vi "Claude_Blit.vi"(0 "Picture":u8[][](array[numeric]), 5 "Sprites":cluster{"Pix":u8[][], "Mask":u8[][]}[](array[cluster]), 7 "State":T2={"Tick"=0, "Phase"=0, "PhaseTicks"=0, "Level"=1, "Room"=0, "X10"=0, "Y10"=0, "VY10"=0, "Mode"=0, "Facing"=0, "Run"=0, "Vert"=0, "StandY"=0, "EntryX10"=0, "EntryY10"=0, "EntryMode"=0, "Lives"=4, "Score"=0, "NextLife"=10000, "KeyR"=0, "KeyB"=0, "KeyY"=0, "Torch"=FALSE, "FloorPhase"=0, "Dead"=FALSE, "LevelStart"=FALSE, "Quit"=FALSE, "Sound"=0, "Seed"=12345, "DemoStep"=0, "Tiles"=[], "World"=[], "Enemies"=[], "Highscores"=[], "Name"=[0, 0, 0], "Cursor"=0}, 9 "View":T1={"Hide"=FALSE, "CX"=0, "CY"=0, "ClaudeIdx"=-1, "ClaudeX"=0, "ClaudeY"=0}, 11 "error in":errorcluster) -> (4 "Picture out":u8[][](array[numeric]), 15 "error out":errorcluster)   [LabVIEW 2020, in "GH_Render.lvlib"]
doc: "Draws Claude (View: ClaudeIdx < 0 hides him) into the screen raster and, while he falls in the treasure room, the parachute above him."
uses:
  GH_Render.lvlib
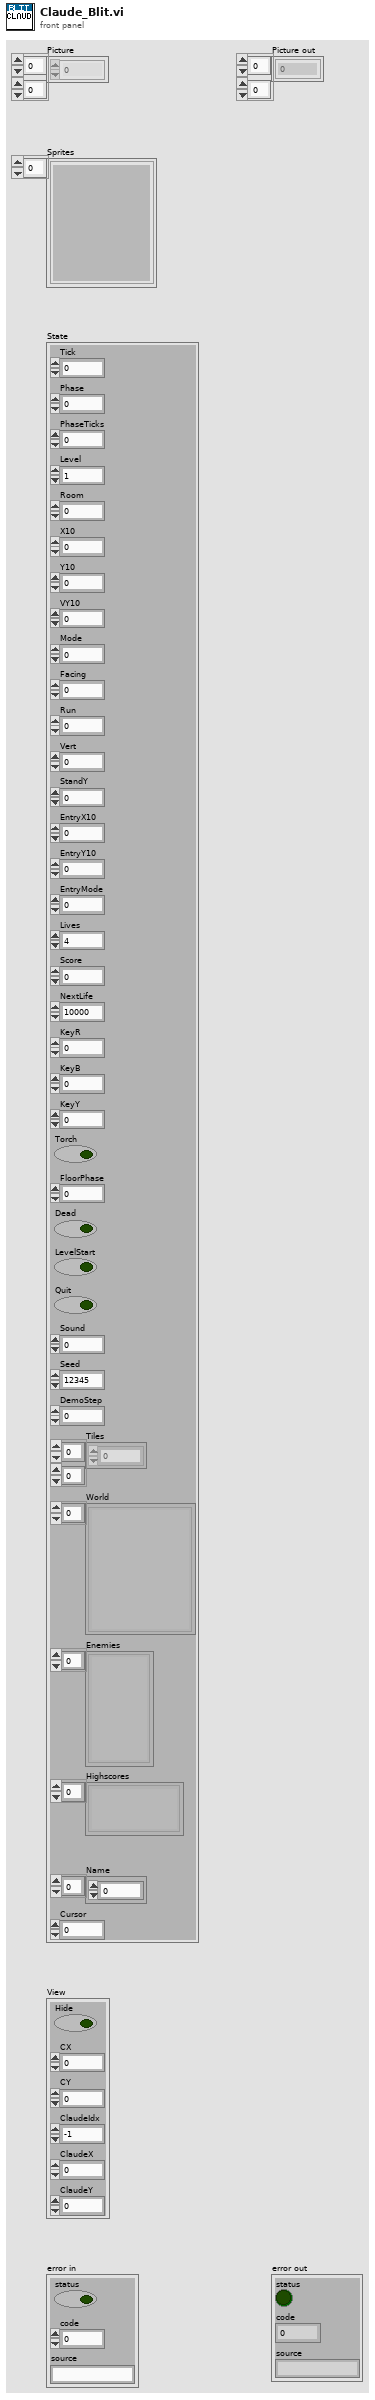
[diagram p1: front panel]
types:
  T1 = cluster{"Hide":bool, "CX":i32, "CY":i32, "ClaudeIdx":i32, "ClaudeX":i32, "ClaudeY":i32}
  T2 = cluster{"Tick":u32, "Phase":i32, "PhaseTicks":i32, "Level":i32, "Room":i32, "X10":i32, "Y10":i32, "VY10":i32, "Mode":i32, "Facing":i32, "Run":i32, "Vert":i32, "StandY":i32, "EntryX10":i32, "EntryY10":i32, "EntryMode":i32, "Lives":i32, "Score":i32, "NextLife":i32, "KeyR":i32, "KeyB":i32, "KeyY":i32, "Torch":bool, "FloorPhase":i32, "Dead":bool, "LevelStart":bool, "Quit":bool, "Sound":i32, "Seed":u32, "DemoStep":i32, "Tiles":u8[][], "World":cluster{"ID":string, "Depth":i32, "Column":i32, "Tiles":u8[][]}[], "Enemies":cluster{"Kind":i32, "X10":i32, "Y10":i32, "Dir":i32, "Mode":i32}[], "Highscores":cluster{"Score":i32, "Name":string}[], "Name":i32[], "Cursor":i32}
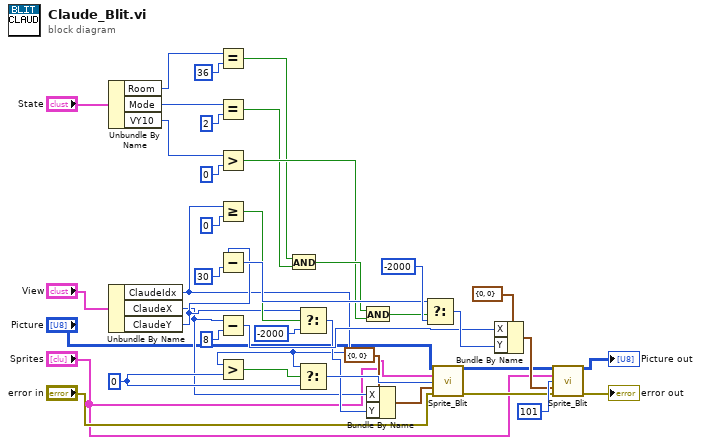
[diagram p0: block diagram]
diagram:
  w15 = 0
  n1 = Unbundle By Name("State") -> ("Room"=w20:i32, "Mode"=w21:i32, "VY10"=w22:i32)
  n2 = Unbundle By Name("View") -> ("ClaudeIdx"=w6:i32, "ClaudeX"=w7:i32, "ClaudeY"=w8:i32)
  n3 = Equal?(x=w20, y=36) -> (x = y?=w24:bool)
  n4 = Equal?(x=w21, y=2) -> (x = y?=w26:bool)
  n5 = Greater?(x=w22, y=0) -> (0:w28:bool)
  n6 = Greater Or Equal?(x=w6, y=0) -> (x >= y?=w11:bool)
  n7 = Subtract(x=w8, y=30) -> (x-y=w35:i32)
  n8 = Subtract(x=w7, y=8) -> (x-y=w33:i32)
  n9 = Greater?(x=w6, y=w15) -> (0:w16:bool)
  n10 = And(x=w24, y=w26) -> (x .and. y?=w29:bool)
  n11 = Select(t=w8, s=w11, f=-2000) -> (s? t:f=w13:i32)
  n12 = Select(t=w6, s=w16, f=w15) -> (s? t:f=w17:i32)
  n13 = And(x=w29, y=w28) -> (x .and. y?=w30:bool)
  n14 = Bundle By Name(cluster=cluster{"X":i32, "Y":i32} {"X"=0, "Y"=0}, "X"=w7, "Y"=w13) -> (w14:cluster{"X":i32, "Y":i32})
  n15 = Select(t=w35, s=w30, f=-2000) -> (s? t:f=w37:i32)
  n16 = call "Sprite_Blit.vi"("Picture"="Picture", "Sprites"="Sprites", "Index"=w17, "Position"=w14, "error in"="error in") -> ("Picture out"=w18:u8[][], "error out"=w19:errorcluster)  [unwired: 9 in]
  n17 = Bundle By Name(cluster=cluster{"X":i32, "Y":i32} {"X"=0, "Y"=0}, "X"=w33, "Y"=w37) -> (w38:cluster{"X":i32, "Y":i32})
  n18 = call "Sprite_Blit.vi"("Picture"=w18, "Sprites"="Sprites", "Index"=101, "Position"=w38, "error in"=w19) -> ("Picture out"=→"Picture out":u8[][], "error out"=→"error out":errorcluster)  [unwired: 9 in]
